vi "Own20261012_AddControlToOwner.vi"() -> ()   [LabVIEW 2024]
panel:
  out "error out":errorcluster caption="错误输出"
  out "object_id":u32
  in  "object_id type":u32
  in  "label":string
  in  "y":i16=100
  in  "x":i16=100
  in  "style":u32
  in  "owner_id":u32
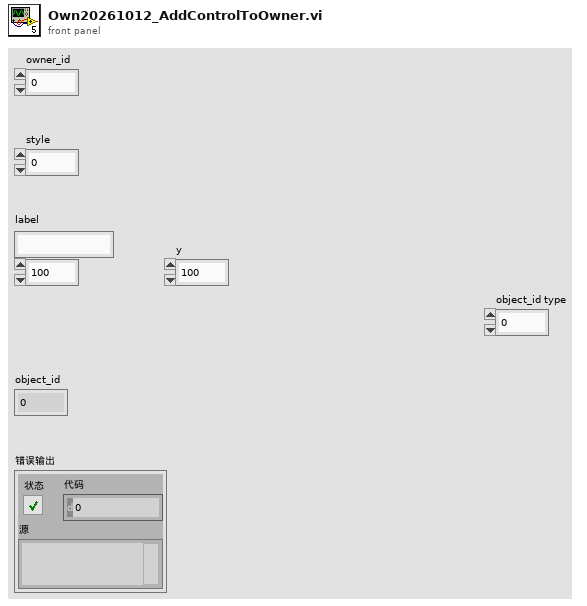
[diagram p1: front panel]
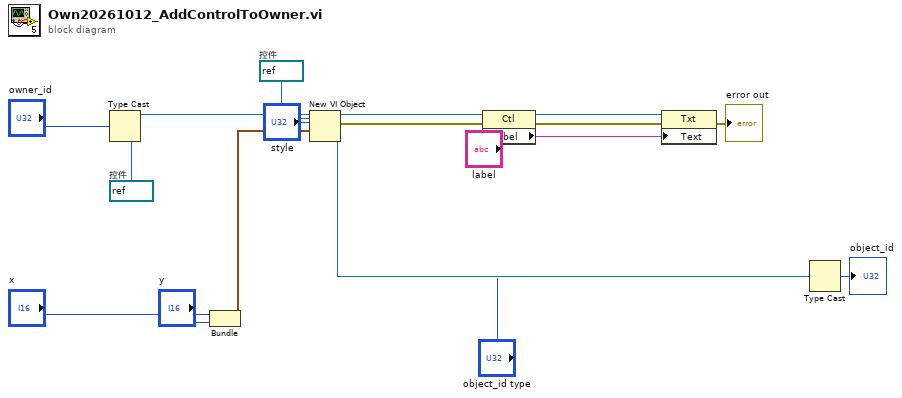
[diagram p0: block diagram]
diagram:
  w14 = refnum<vi> refnum  # 控件
  w15 = refnum<vi> refnum  # 控件
  n1 = Type Cast ("强制类型转换")(type=w15, x="owner_id") -> (*(type *) &x=w13:refnum<vi>)
  n2 = Bundle ("捆绑")("x"="x", "y"="y") -> (w9:cluster{"x":i16, "y":i16})  [unwired: 1 in]
  n3 = New VI Object ("新建VI对象")(vi object class=w14, owner refnum=w13, style="style", position/next to=w9) -> (object refnum=w8:refnum<vi>, 0:w5:errorcluster)  [unwired: 4 in]
  n4 = property on="属性节点" class="Ctl"(reference=w8, error in=w5) -> (error out=w4:errorcluster, "Label"=w7:refnum<vi>)  [unwired: 1 out]
  n5 = property on="属性节点" class="Txt"(reference=w7, error in=w4, "Text"="label") -> (error out=→"error out":errorcluster)  [unwired: 1 out]
  n6 = Type Cast ("强制类型转换")(type="object_id type", x=w8) -> (*(type *) &x=→"object_id":u32)
